vi "user32 GetWindowThreadProcessId.vi"(0 "hWnd":u64, 11 "error in":errorcluster) -> (4 "process ID":u32, 6 "thread ID":u32, 15 "error out":errorcluster)   [LabVIEW 2020, in "RemoteVI.lvlib"]
doc: "Returns the thread and the process that created the window hWnd, through user32.dll GetWindowThreadProcessId (stdcall, called in any thread). Both are 0 when hWnd is not a window. When error in carries an error the DLL is not called. Generated by scripts\\Build Win32 Wrappers.vi - do not edit by hand, rebuild it."
uses:
  RemoteVI.lvlib
  user32.dll
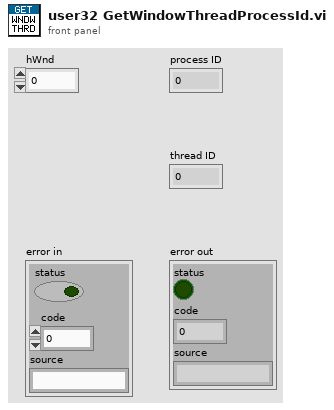
[diagram p1: front panel]
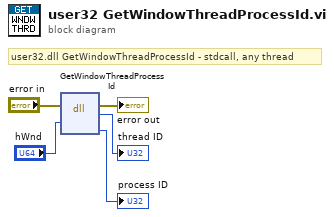
[diagram p0: block diagram]
diagram:
  # "user32.dll GetWindowThreadProcessId - stdcall, any thread"
  n1 = dll-call lib="user32.dll" fn="GetWindowThreadProcessId"(error in="error in", "hWnd"="hWnd") -> (error out=→"error out":errorcluster, →"thread ID":u32, "lpdwProcessId"=→"process ID":u32)  [unwired: 4 in, 1 out]
